vi "test labview version.vi"(8 "error in (no error)":errorcluster) -> (0 "error out":errorcluster, 3 "body":string)   [LabVIEW 2020, in "MCP Server tests.lvlib"]
doc: "serverInfo.additionalDetails.labviewVersion in the initialize result is the version of the LabVIEW that runs the server (application property Version Number)."
uses:
  MCP Server tests.lvlib
  c5478510-6237-4867-93d3-3b997bc085be.vi
  <vilib>/JDP Science/JSONtext/Next JSON Value.vi
  <vilib>/JDP Science/JSONtext/String Subset.vi
  <vilib>/JDP Science/JSONtext/Parsing/Advance past next JSON Value (inlined COPY).vi
  <vilib>/JDP Science/JSONtext/Parsing/Advance past whitespace.vi
  <vilib>/JDP Science/JSONtext/Parsing/Advance past String.vi
  <vilib>/JDP Science/JSONtext/Parsing/Advance past Number.vi
  <vilib>/JDP Science/JSONtext/Parsing/Advance past Line Ending.vi
  <vilib>/JDP Science/JSONtext/Parsing/Parse Full Path or Item Name.vi
  <vilib>/JDP Science/JSONtext/Parsing/Advance past Array.vi
  <vilib>/JDP Science/JSONtext/Parsing/Advance past Object.vi
  <vilib>/JDP Science/JSONtext/support/Error Cluster From Code.vi
  <vilib>/JDP Science/JSONtext/Offset/Find Item Locations by Path.vi
  <vilib>/JDP Science/JSONtext/JSON text to Variant.vi
  <vilib>/JDP Science/JSONtext/LVClass Serializer/JSONtext LVClass Serializer.lvclass
  <vilib>/addons/_JKI Toolkits/Caraya/classes/Test/Test.lvclass
  <vilib>/JDP Science/JSONtext/JSONtext.lvlib
  <vilib>/addons/_JKI Toolkits/Caraya/classes/Assert/Assert.lvclass
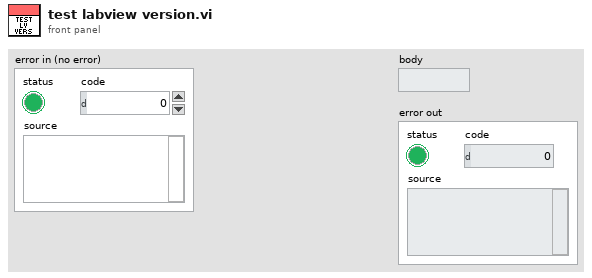
[diagram p1: front panel]
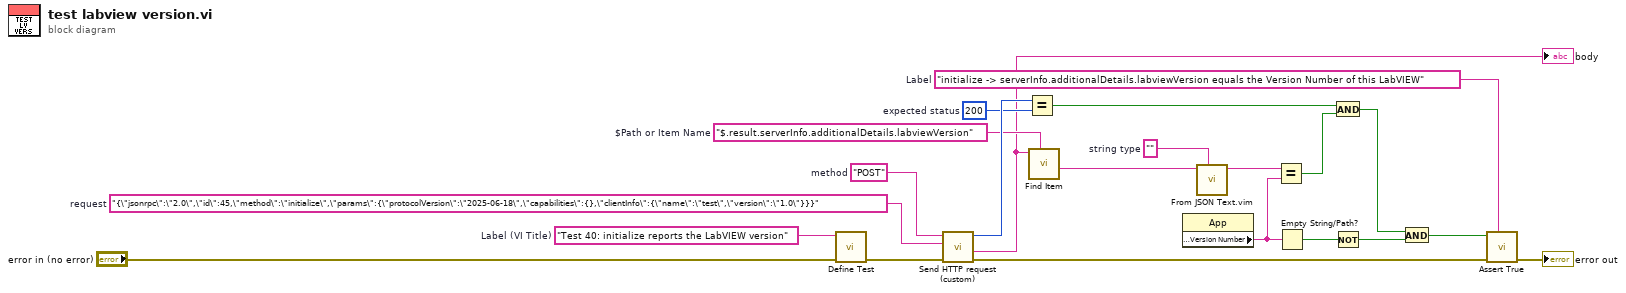
[diagram p0: block diagram]
diagram:
  w3 = "initialize -> serverInfo.additionalDetails.labviewVersion equals the Version Number of this LabVIEW"  # Label
  w13 = ""  # string type
  w15 = "$.result.serverInfo.additionalDetails.labviewVersion"  # $Path or Item Name
  w16 = 200  # expected status
  w19 = "{\"jsonrpc\":\"2.0\",\"id\":45,\"method\":\"initialize\",\"params\":{\"protocolVersion\":\"2025-06-18\",\"capabilities\":{},\"clientInfo\":{\"name\":\"test\",\"version\":\"1.0\"}}}"  # request
  w20 = "POST"  # method
  w22 = "Test 40: initialize reports the LabVIEW version"  # Label (VI Title)
  n1 = call <vilib>:"Define Test.vi"("error in (no error)"="error in (no error)", "Label (VI Title)"=w22) -> ("error out"=w18:errorcluster)  [unwired: 8 in, 1 out]
  n2 = call "Send HTTP request (custom).vi"("error in (no error)"=w18, "request"=w19, "method"=w20) -> ("error out"=w4:errorcluster, "response"=w2:string, "status code"=w17:i32)  [unwired: 5 in, 1 out]
  "body" <- w2
  n3 = Equal?(x=w17, y=w16) -> (x = y?=w9:bool)
  n4 = call <vilib>:"Find Item.vi"("$Path or Item Name"=w15, "JSON"=w2) -> ("<JSON>"=w14:string)  [unwired: 6 in, 3 out]
  n5 = property class="App"() -> ("Application:Version Number"=w11:string)  [unwired: 2 in, 2 out]
  n6 = call "From JSON Text.vim"("Data Type and Default Value"=w13, "JSON"=w14) -> ("Data out"=w12:string)  [unwired: 8 in, 1 out]
  n7 = Equal?(x=w12, y=w11) -> (x = y?=w8:bool)
  n8 = Empty String/Path?(string/path=w11) -> (empty?=w10:bool)
  n9 = And(x=w9, y=w8) -> (x .and. y?=w7:bool)
  n10 = Not(x=w10) -> (.not. x?=w6:bool)
  n11 = And(x=w7, y=w6) -> (x .and. y?=w5:bool)
  n12 = call <vilib>:"Assert True.vi"("Label"=w3, "error in (no error)"=w4, "True?"=w5) -> ("error out"=→"error out":errorcluster)  [unwired: 7 in, 1 out]
